vi "Destroy.vi"(0 "reference in":refnum<class "G4SubTemplate_Simple_6x8x6.lvclass">, 5 "Error In":errorcluster) -> (14 "reference out":refnum<class "G4SubTemplate_Simple_6x8x6.lvclass">, 19 "Error Out":errorcluster)   [LabVIEW 2020, in "G4SubTemplate_Simple_6x8x6.lvclass"]
uses:
  G4SubTemplate_Simple_6x8x6.lvclass
  G4BaseTemplate_Simple_6x8x6/G4BaseTemplate_Simple_6x8x6.lvclass
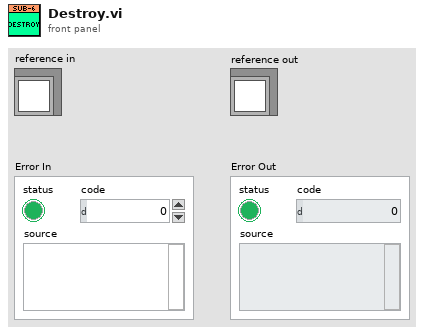
[diagram p1: front panel]
types:
  T1 = typedef "G4BaseTemplate_Simple_6x8x6.lvclass/ObjectAttributes.ctl" = cluster{"Attribute1":dbl}
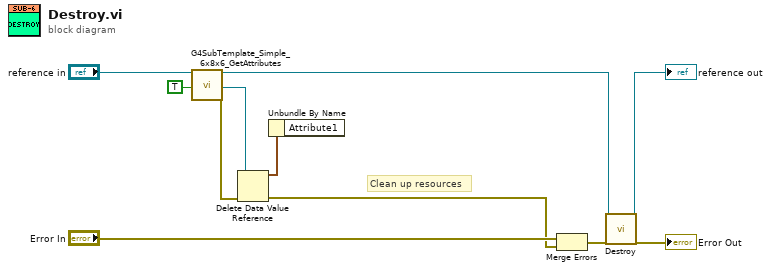
[diagram p0: block diagram]
diagram:
  # "Clean up resources"
  n1 = call "G4SubTemplate_Simple_6x8x6_GetAttributes.vi"("reference in"="reference in", "OnlyGetDvrReference(False)"=TRUE) -> ("reference out"=w6:refnum<class "G4SubTemplate_Simple_6x8x6.lvclass">, "DataRef"=w9:refnum<data-value>, "Error Out"=w10:errorcluster)  [unwired: 14 in, 1 out]
  n2 = Delete Data Value Reference(data value reference=w9, error in=w10) -> (data value=w1:T1, error out=w3:errorcluster)
  n3 = Unbundle By Name(w1) -> ()  [unwired: 1 out]
  n4 = Merge Errors("Error In", w3) -> (w8:errorcluster)
  n5 = call-parent "Destroy.vi"("reference in"=w6, "Error In"=w8) -> ("reference out"=→"reference out":refnum<class "G4SubTemplate_Simple_6x8x6.lvclass">, "Error Out"=→"Error Out":errorcluster)  [unwired: 16 in]
